vi "ASDE Burst Region Data Pass Formation Modified VI.vi"(4 "B#":i32, 5 "A New folder":string, 6 "Burst Time (ms)":string="3.12", 7 "Burst End":string="3.12", 8 "error in":errorcluster, 9 "Burst Start":string="3.12", 10 "N #":string="3.12", 11 "Filename":path) -> (0 "error out":errorcluster, 3 "BSX Pass":path)   [LabVIEW 2018]
panel:
  out "取り除かれたパス 2":path
  out "取り除かれたパス":path
  out "BS? 3":bool caption="既存するファイルまたはフォルダ?"
  in  "AInfo":string
  out "BS? 2":bool caption="既存するファイルまたはフォルダ?"
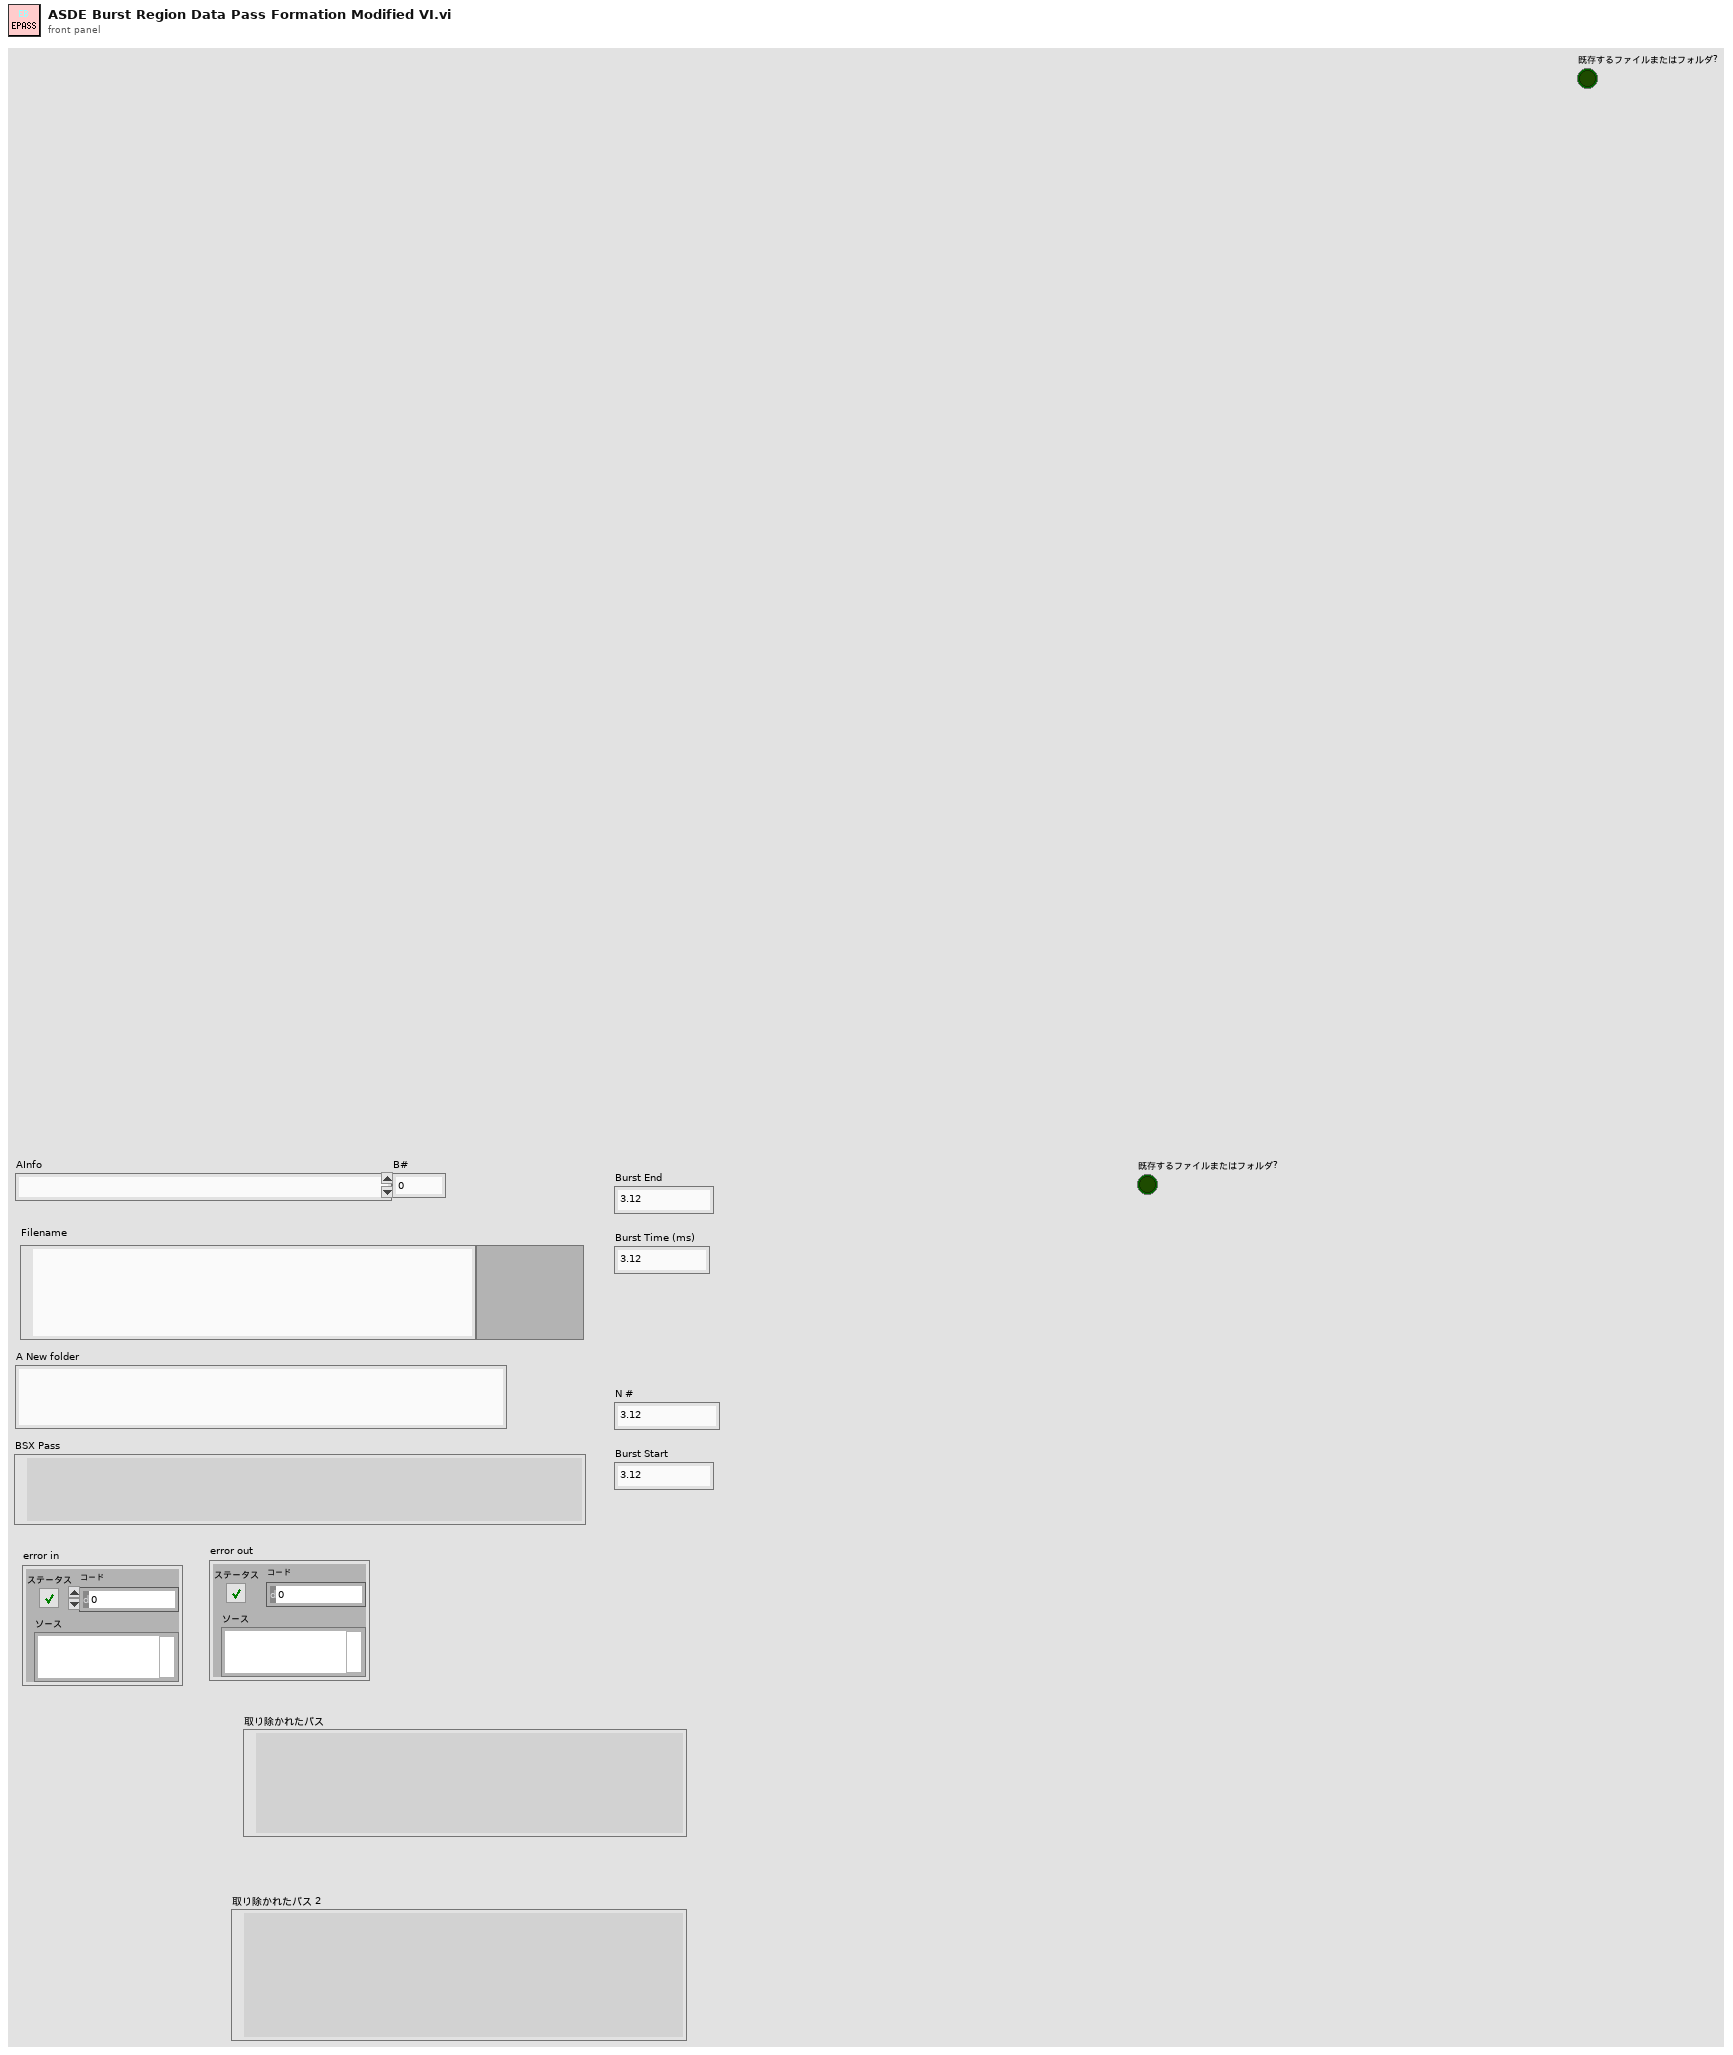
[diagram p1: front panel]
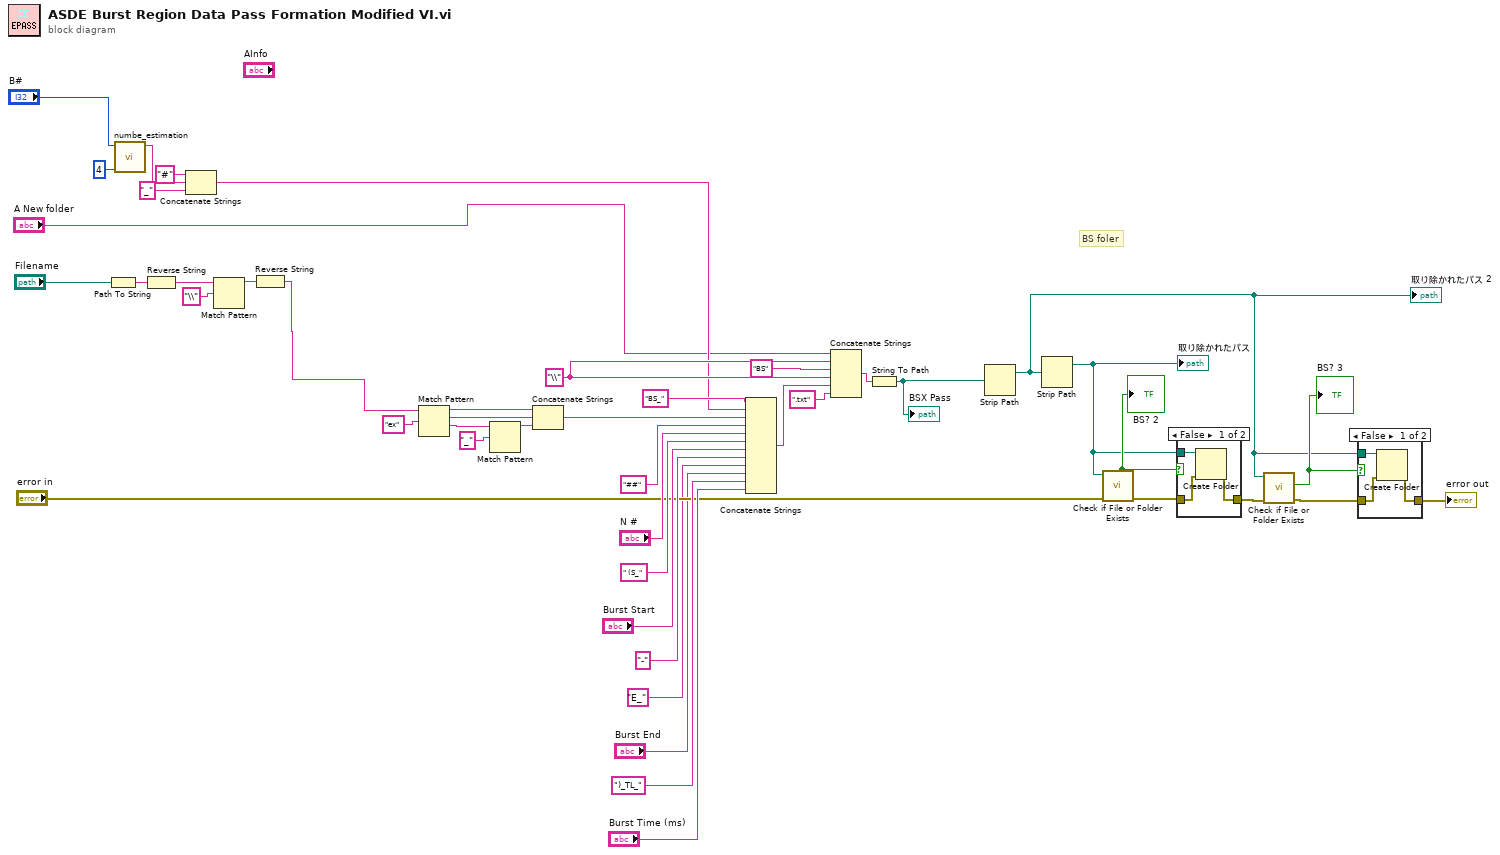
[diagram p0: block diagram]
diagram:
  w12 = "\\" ("検索文字列")
  # "BS foler"
  n1 = Path To String(path="Filename") -> (string=w42:string)
  n2 = call "numbe_estimation.vi"("桁数"=4, "数値"="B#") -> ("数値文字列"=w5:string)  [unwired: 9 in]
  n3 = Reverse String(1:w42) -> (0:w44:string)
  n4 = Concatenate Strings("#" ("文字列"), w5, "_" ("文字列")) -> (w3:string)
  n5 = Match Pattern(string=w44, regular expression="\\" ("検索文字列")) -> (before substring=w43:string)  [unwired: 1 in, 3 out]
  n6 = Reverse String(1:w43) -> (0:w38:string)
  n7 = Match Pattern(string=w38, regular expression="ex" ("正規表現")) -> (before substring=w34:string, match substring=w33:string, after substring=w35:string)  [unwired: 1 in, 1 out]
  n8 = Match Pattern(string=w35, regular expression="_" ("正規表現")) -> (before substring=w32:string)  [unwired: 1 in, 3 out]
  n9 = Concatenate Strings(w34, w33, w32) -> (w27:string)
  n10 = Concatenate Strings("BS_" ("文字列"), w3, w27, "##" ("文字列"), "N #", " (S_" ("文字列"), "Burst Start", "-" ("文字列"), "E_" ("文字列"), "Burst End", ")_TL_" ("文字列"), "Burst Time (ms)") -> (w31:string)
  n11 = Concatenate Strings("A New folder", w12, "BS" ("文字列"), w12, w31, ".txt" ("連結文字列")) -> (w29:string)
  n12 = String To Path(string=w29) -> (path=w28:path)
  "BSX Pass" <- w28
  n13 = Strip Path(path=w28) -> (stripped path=w15:path)  [unwired: 1 out]
  "取り除かれたパス 2" <- w15
  n14 = Strip Path(path=w15) -> (stripped path=w20:path)  [unwired: 1 out]
  "取り除かれたパス" <- w20
  n15 = call <vilib>:"Check if File or Folder Exists.vi"("error in (no error)"="error in", "path"=w20) -> ("error out"=w13:errorcluster, "file or folder exists?"=w21:bool)  [unwired: 7 in, 1 out]
  "BS? 2" <- w21
  n16 = case shown="False" w21 {
    tunnel: w20 -> [w48 _]
    tunnel: w13 -> [w47 w49]
    tunnel: [w46 w49] -> w18
    frame False {
      n17 = Create Folder(path (use dialog)=w48, error in=w47) -> (error out=w46:errorcluster)  [unwired: 1 in, 2 out]
    }
    frame True {
    }
  }
  n18 = call <vilib>:"Check if File or Folder Exists.vi"("error in (no error)"=w18, "path"=w15) -> ("error out"=w17:errorcluster, "file or folder exists?"=w19:bool)  [unwired: 7 in, 1 out]
  "BS? 3" <- w19
  n19 = case shown="False" w19 {
    tunnel: w15 -> [w52 _]
    tunnel: w17 -> [w51 w53]
    tunnel: [w50 w53] -> w16
    frame False {
      n20 = Create Folder(path (use dialog)=w52, error in=w51) -> (error out=w50:errorcluster)  [unwired: 1 in, 2 out]
    }
    frame True {
    }
  }
  "error out" <- w16
